vi "VIH Utility - FILE - Get and Replace Extension (File Name).vi"(10 "new extension (none)":string, 11 "File name":string) -> (2 "extension":string, 3 "File name out":string)   [LabVIEW 2014]
doc: "::: VI Helpeks :::\nCopyright (c) 2000-2026 Konstantin Shifershteyn. All rights reserved."
panel:
  # "VI Helpeks\nCopyright (c) 2012-2026 Konstantin Shifershteyn"
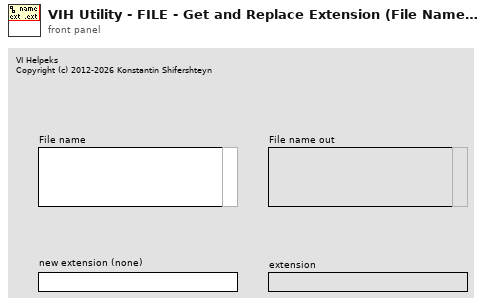
[diagram p1: front panel]
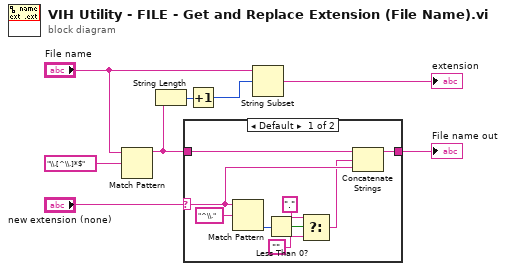
[diagram p0: block diagram]
diagram:
  n1 = Match Pattern(string="File name", regular expression="\\.[^\\.]*$") -> (before substring=w4:string)  [unwired: 4 out]
  n2 = String Length(string=w4) -> (length=w5:i32)
  n3 = case shown="Default" "new extension (none)" {
    selector: "new extension (none)" -> [w15 _]
    tunnel: w4 -> [w16 w18]
    tunnel: [w9 w18] -> w2
    frame Default {
      n4 = Match Pattern(string=w15, regular expression="^\\.") -> (offset past match=w14:i32)  [unwired: 4 out]
      n5 = Less Than 0?(x=w14) -> (x < 0?=w13:bool)
      n6 = Select(t=".", s=w13, f="") -> (s? t:f=w10:string)
      n7 = Concatenate Strings(w16, w10, w15) -> (w9:string)
    }
    frame "" {
    }
  }
  "File name out" <- w2
  n8 = Increment(x=w5) -> (x+1=w3:i32)
  n9 = String Subset(string="File name", offset (0)=w3) -> (substring=→"extension":string)  [unwired: 1 out]
